vi "SC Choose Project.vi"(9 "projects":T1(array[cluster]), 10 "window title":string="Choose a Project", 11 "selected":i32) -> (1 "index":i32=-1, 2 "chosen?":bool)   [LabVIEW 2023]
doc: "Shows a window listing the robot's projects (bold: the one it runs; italics: no local copy on this computer) with OK and Cancel buttons, the selected one chosen first. Double-clicking an item or selecting it and clicking OK returns its index; chosen? is false when the user cancels or closes the window."
panel:
  in  "Cancel":bool
  in  "OK":bool
  in  "Projects on the robot":i32(listbox)
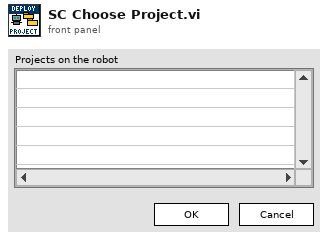
[diagram p1: front panel]
types:
  T1 = cluster{"name":string, "running":bool, "local copy":bool}[]
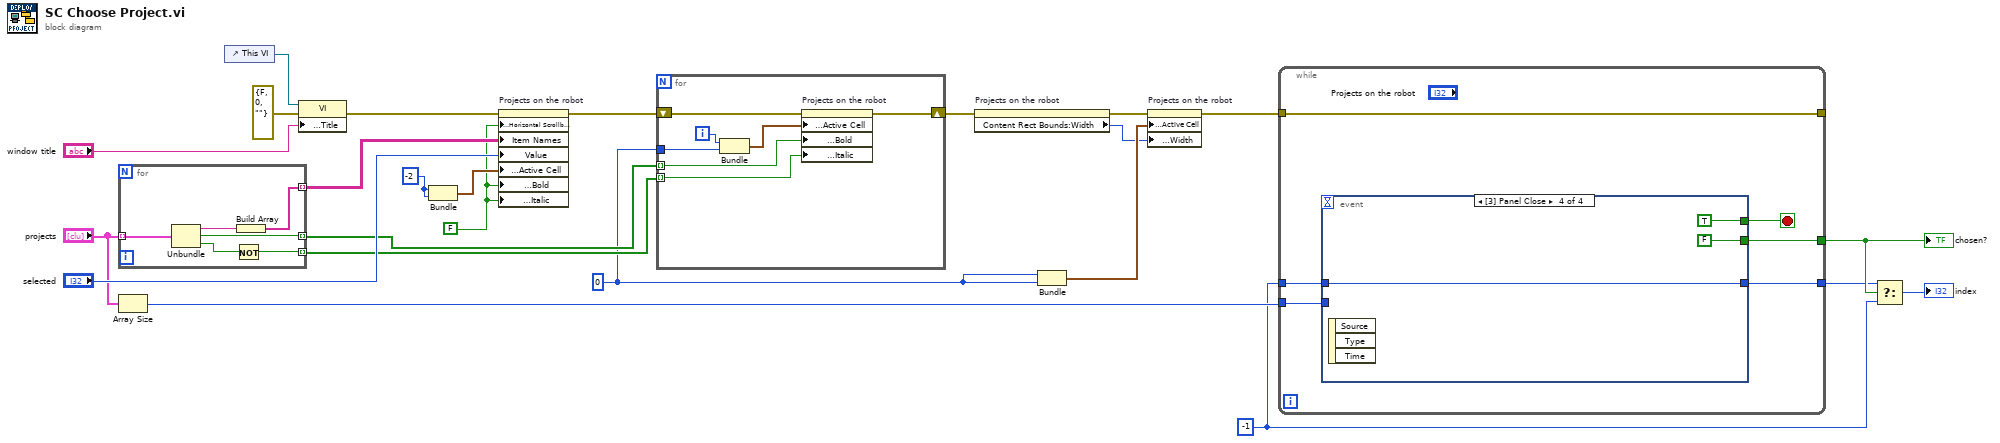
[diagram p0: block diagram]
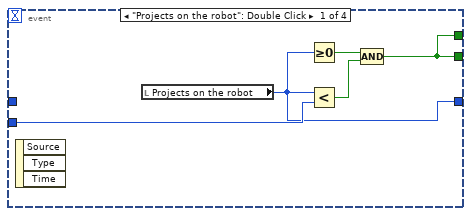
[diagram p2: hidden frame]
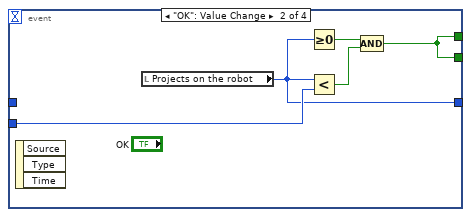
[diagram p3: hidden frame]
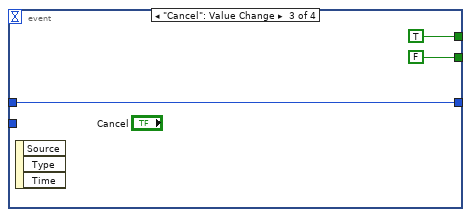
[diagram p4: hidden frame]
diagram:
  w16 = FALSE
  w11 = 0
  w21 = -2
  w2 = -1
  n1 = for {
    tunnel: "projects" -> [w30] mode=indexing
    tunnel: [w27] -> w18 mode=indexing
    tunnel: [w26] -> w15 mode=indexing
    tunnel: [w25] -> w14 mode=indexing
    n2 = Unbundle(w30) -> ("name"=w29:string, "running"=w26:bool, "local copy"=w28:bool)
    n3 = Not(x=w28) -> (.not. x?=w25:bool)
    n4 = Build Array(w29) -> (w27:string[])
  }
  n5 = Array Size(array="projects") -> (size(s)=w6:i32)
  n6 = control-ref of="This VI"() -> (w24:refnum<vi>)
  n7 = property class="VI"(reference=w24, error in=errorcluster {"status"=FALSE, "code"=0, "source"=""}, "Front Panel Window:Title"="window title") -> (error out=w20:errorcluster)  [unwired: 1 out]
  n8 = Bundle(w21, w21) -> (w17:cluster{i32, i32})  [unwired: 1 in]
  n9 = property on="Projects on the robot" class="MCListbox (strict)"(error in=w20, "Visible Items:Horizontal Scrollbar Visible"=w16, "Item Names"=w18, "Value"="selected", "Active Cell:Active Cell"=w17, "Active Cell:Cell Font:Bold"=w16, "Active Cell:Cell Font:Italic"=w16) -> (error out=w13:errorcluster)  [unwired: 1 in, 1 out]
  n10 = for {
    tunnel: w15 -> [w34] mode=indexing
    tunnel: w14 -> [w33] mode=indexing
    tunnel: w11 -> [w37]
    shift-right: [w32] -> w12
    shift-left: w13 -> [w36]
    i -> [w31]
    n11 = Bundle(w31, w37) -> (w35:cluster{i32, i32})  [unwired: 1 in]
    n12 = property on="Projects on the robot" class="MCListbox (strict)"(error in=w36, "Active Cell:Active Cell"=w35, "Active Cell:Cell Font:Bold"=w34, "Active Cell:Cell Font:Italic"=w33) -> (error out=w32:errorcluster)  [unwired: 1 in, 1 out]
  }
  n13 = property on="Projects on the robot" class="MCListbox (strict)"(error in=w12) -> (error out=w10:errorcluster, "Content Rect Bounds:Width"=w8:i32)  [unwired: 1 in, 1 out]
  n14 = Bundle(w11, w11) -> (w9:cluster{i32, i32})  [unwired: 1 in]
  n15 = property on="Projects on the robot" class="MCListbox (strict)"(error in=w10, "Active Cell:Active Cell"=w9, "Active Cell:Cell Size:Width"=w8) -> (error out=w5:errorcluster)  [unwired: 1 in, 1 out]
  n16 = while {
    tunnel: w6 -> [w42]
    tunnel: w5 -> [w43]
    tunnel: w2 -> [w41]
    tunnel: [w40] -> w4
    tunnel: [w39] -> w3
    tunnel: [w43] -> _
    stop <- w38 stop-if-true
    n17 = event shown="[3] Panel Close" {
      selector: _ -> [_ _ _ _]
      dyn-events: _ -> [_ _ _ _]
      timeout: _ -> [_ _ _ _]
      tunnel: w42 -> [w48 w53 _ _]
      tunnel: w41 -> [_ _ w54 w57]
      tunnel: [w45 w50 TRUE TRUE] -> w38
      tunnel: [w45 w50 FALSE FALSE] -> w40
      tunnel: [w44 w49 w54 w57] -> w39
      event "Projects on the robot": Double Click {
        n18 = event-data() -> ()  [unwired: 1 in, 3 out]
        n19 = local read "Projects on the robot"() -> (w44:i32)
        n20 = Greater Or Equal To 0?(x=w44) -> (x >= 0?=w47:bool)
        n21 = Less?(x=w44, y=w48) -> (x < y?=w46:bool)
        n22 = Compound Arithmetic op=AND(w47, w46) -> (w45:bool)
      }
      event "OK": Value Change {
        n23 = event-data() -> ()  [unwired: 1 in, 3 out]
        n24 = local read "Projects on the robot"() -> (w49:i32)
        n25 = Greater Or Equal To 0?(x=w49) -> (x >= 0?=w52:bool)
        n26 = Less?(x=w49, y=w53) -> (x < y?=w51:bool)
        n27 = Compound Arithmetic op=AND(w52, w51) -> (w50:bool)
      }
      event "Cancel": Value Change {
        n28 = event-data() -> ()  [unwired: 1 in, 3 out]
      }
      event Panel Close {
        n29 = event-data() -> ()  [unwired: 1 in, 3 out]
      }
    }
  }
  "chosen?" <- w4
  n30 = Select(t=w3, s=w4, f=w2) -> (s? t:f=→"index":i32)
